vi "Posicions aleatories.vi"() -> (2 "x":dbl, 3 "y":dbl)   [LabVIEW 2023]
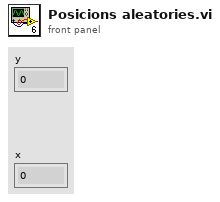
[diagram p1: front panel]
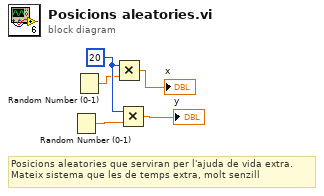
[diagram p0: block diagram]
diagram:
  w3 = 20
  # "Posicions aleatories que serviran per l'ajuda de vida extra. \nMateix sistema que les de temps extra, molt senzill"
  n1 = Random Number (0-1)() -> (number: 0 to 1=w1:dbl)
  n2 = Random Number (0-1)() -> (number: 0 to 1=w2:dbl)
  n3 = Multiply(x=w3, y=w2) -> (x*y=→"x":dbl)
  n4 = Multiply(x=w3, y=w1) -> (x*y=→"y":dbl)
